vi "Set Description.vi"(8 "error in":errorcluster, 11 "ILabVIEWFile in":refnum<class "LabVIEW File.lvclass">) -> (0 "error out":errorcluster, 3 "ILabVIEWFile out":refnum<class "LabVIEW File.lvclass">)   [LabVIEW 2026, in "LabVIEW File.lvclass"]
doc: "Set description of labview file (vi or type definition)."
uses:
  LabVIEW File.lvclass
  LabVIEW File.lvclass/LabVIEW File.ctl
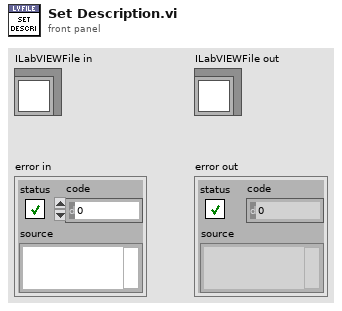
[diagram p1: front panel]
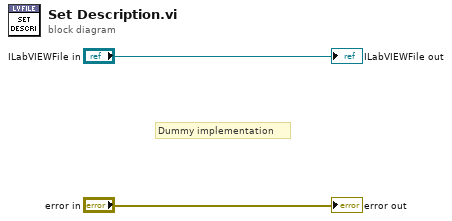
[diagram p0: block diagram]
diagram:
  # "Dummy implementation"
  "error out" <- "error in"
  "ILabVIEWFile out" <- "ILabVIEWFile in"
